vi "1g_v3.vi"() -> ()   [LabVIEW 2017]
uses:
  <vilib>/Instr/_visa.llb/VISA Configure Serial Port (Instr).vi
panel:
  in  "stop":bool
  out "return count 2":u32
  out "read buffer 2":string
  out "return count":u32
  out "read buffer":string
  in  "milliseconds":dbl=100.0 min=100.0
  out "XY Graph":cluster{dbl[], u16[]}(graph)
  out "VISA resource name out":refnum<visa-resource-name>
  in  "VISA resource name":refnum<visa-resource-name>="COM3" caption="Serial COM port"
  # "Partially working code"
  # "REAL TIME FIBER OPTIC TEMPERATURE MONITORING SYSTEM"
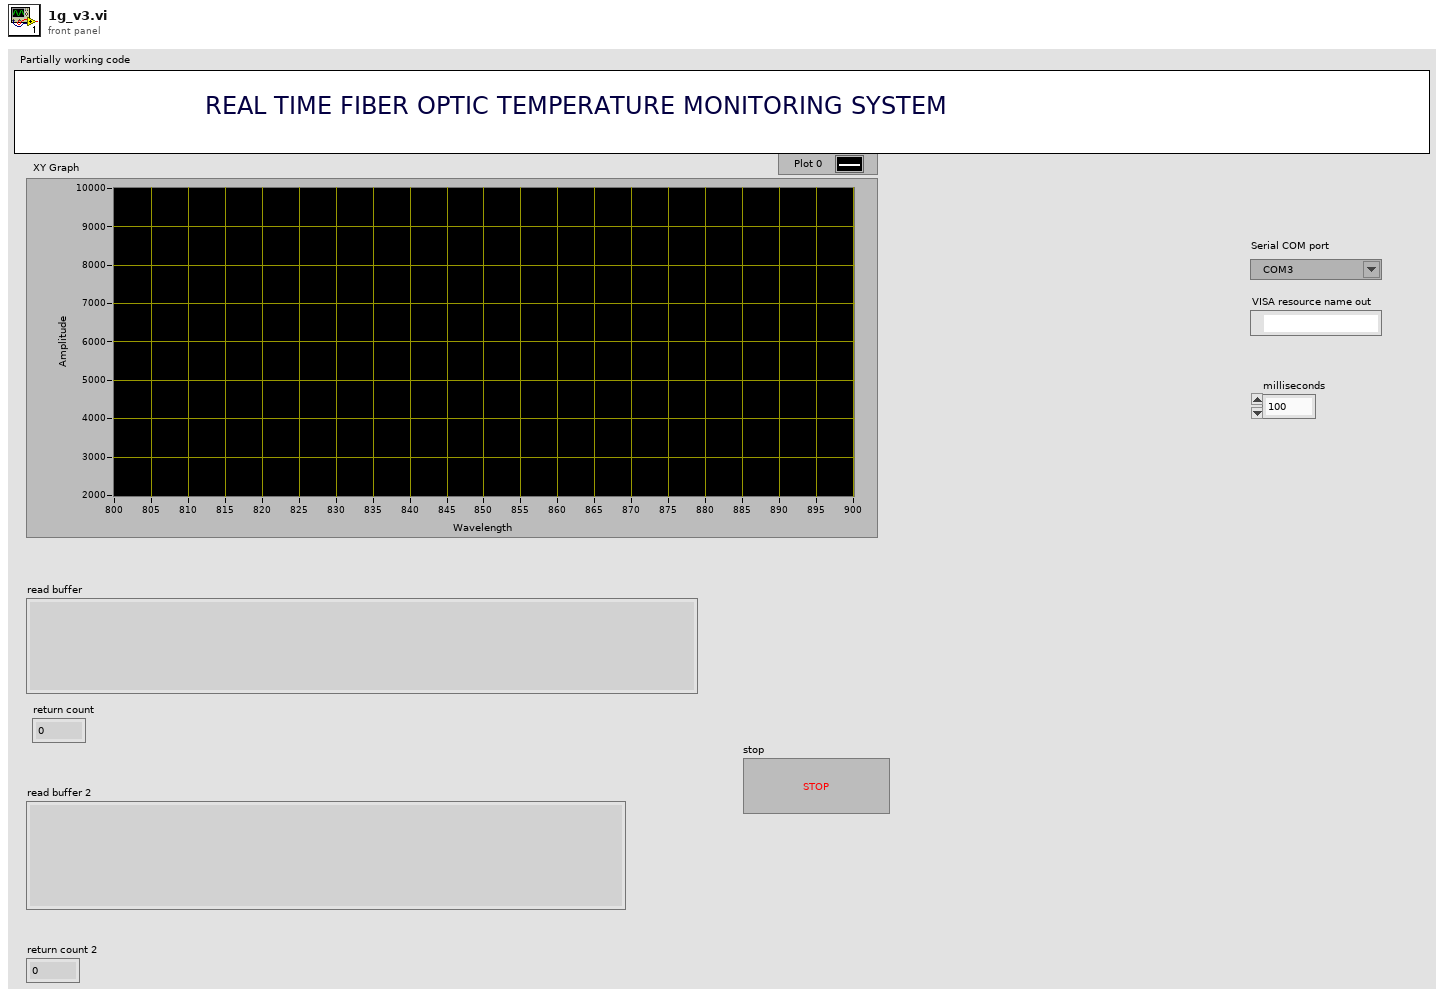
[diagram p1: front panel]
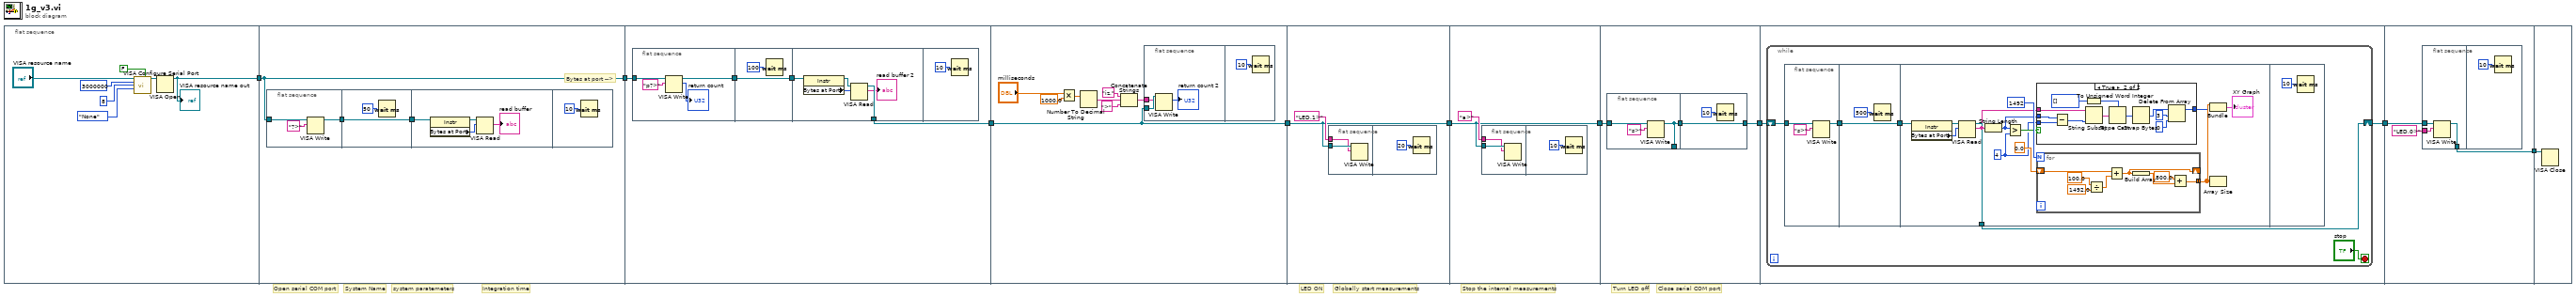
[diagram p0: block diagram]
diagram:
  # "Globally start measurements"
  # "LED ON"
  # "System Name"
  # "Integration time"
  # "system paratemeters"
  # "Close serial COM port"
  # "Turn LED off"
  # "Stop the internal measurements"
  # "Open serial COM port"
  n1 = flat-sequence {
    tunnel: [w10] -> w3
    tunnel: [w17] -> w9
    tunnel: w3 -> [w17]
    tunnel: w9 -> [w31]
    tunnel: [w30] -> w8
    tunnel: w8 -> [w49]
    tunnel: [w49] -> w7
    tunnel: w7 -> [w58]
    tunnel: [w58] -> w4
    tunnel: [w63] -> w2
    tunnel: w4 -> [w63]
    tunnel: w2 -> [w70]
    tunnel: [w68] -> w1
    tunnel: [w77] -> w6
    tunnel: w1 -> [w76]
    tunnel: w6 -> [w123]
    tunnel: [w122] -> w5
    tunnel: w5 -> [w129]
    frame #0 {
      n2 = call-poly "VISA Configure Serial Port"("VISA resource name"="VISA resource name", "Enable Termination\nChar (T)"=FALSE ("Enable Termination\nChar (T)"), "baud rate (9600)"=u32 3000000, "data bits (8)"=u16 8, "parity (0:none)"=enum16{"None", "Odd", "Even", "Mark", "Space"}."None") -> ("VISA resource name out"=w16:refnum<visa-resource-name>)  [unwired: 9 in, 1 out]
      n3 = VISA Open(VISA resource name=w16) -> (VISA resource name=w10:refnum<visa-resource-name>)  [unwired: 4 in, 1 out]
      "VISA resource name out" <- w10
    }
    frame #1 {
      # "Bytes at port -->"
      n4 = flat-sequence {
        tunnel: [w22] -> w19
        tunnel: w17 -> [w21]
        tunnel: [w23] -> w18
        tunnel: w19 -> [w23]
        tunnel: w18 -> [w28]
        frame #0 {
          n5 = VISA Write(VISA resource name=w21, write buffer="?>") -> (VISA resource name out=w22:refnum<visa-resource-name>)  [unwired: 1 in, 2 out]
        }
        frame #1 {
          n6 = Wait (ms)(milliseconds to wait=u32 50 ("Zu wartende ms")) -> ()  [unwired: 1 out]
        }
        frame #2 {
          n7 = property class="Instr"(reference=w28) -> (reference out=w27:refnum<visa-resource-name>, "Bytes at Port"=w26:u32)  [unwired: 1 in, 1 out]
          n8 = VISA Read(VISA resource name=w27, byte count=w26) -> (read buffer=→"read buffer":string)  [unwired: 1 in, 3 out]
        }
        frame #3 {
          n9 = Wait (ms)(milliseconds to wait=u32 10 ("Zu wartende ms")) -> ()  [unwired: 1 out]
        }
      }
    }
    frame #2 {
      n10 = flat-sequence {
        tunnel: [w37] -> w33
        tunnel: w31 -> [w35]
        tunnel: [w38] -> w32
        tunnel: w33 -> [w38]
        tunnel: w32 -> [w44]
        tunnel: [w41] -> w30
        frame #0 {
          n11 = VISA Write(VISA resource name=w35, write buffer="p?>") -> (VISA resource name out=w37:refnum<visa-resource-name>, return count=→"return count":u32)  [unwired: 1 in, 1 out]
        }
        frame #1 {
          n12 = Wait (ms)(milliseconds to wait=u32 100 ("Zu wartende ms")) -> ()  [unwired: 1 out]
        }
        frame #2 {
          n13 = property class="Instr"(reference=w44) -> (reference out=w43:refnum<visa-resource-name>, "Bytes at Port"=w42:u32)  [unwired: 1 in, 1 out]
          n14 = VISA Read(VISA resource name=w43, byte count=w42) -> (VISA resource name out=w41:refnum<visa-resource-name>, read buffer=→"read buffer 2":string)  [unwired: 1 in, 2 out]
        }
        frame #3 {
          n15 = Wait (ms)(milliseconds to wait=u32 10 ("Zu wartende ms")) -> ()  [unwired: 1 out]
        }
      }
    }
    frame #3 {
      n16 = Multiply(x="milliseconds", y=1000.0) -> (x*y=w46:dbl)
      n17 = Number To Decimal String(number=w46) -> (decimal integer string=w53:string)  [unwired: 1 in]
      n18 = Concatenate Strings("iz," ("String"), w53, ">" ("String")) -> (w50:string)
      n19 = flat-sequence {
        tunnel: w49 -> [w56]
        tunnel: w50 -> [w55]
        frame #0 {
          n20 = VISA Write(VISA resource name=w56, write buffer=w55) -> (return count=→"return count 2":u32)  [unwired: 1 in, 2 out]
        }
        frame #1 {
          n21 = Wait (ms)(milliseconds to wait=u32 10 ("Zu wartende ms")) -> ()  [unwired: 1 out]
        }
      }
    }
    frame #4 {
      n22 = flat-sequence {
        tunnel: w58 -> [w61]
        tunnel: "LED,1>" ("String") -> [w60]
        frame #0 {
          n23 = VISA Write(VISA resource name=w61, write buffer=w60) -> ()  [unwired: 1 in, 3 out]
        }
        frame #1 {
          n24 = Wait (ms)(milliseconds to wait=u32 20 ("Zu wartende ms")) -> ()  [unwired: 1 out]
        }
      }
    }
    frame #5 {
      n25 = flat-sequence {
        tunnel: w63 -> [w66]
        tunnel: "a>" ("String") -> [w65]
        frame #0 {
          n26 = VISA Write(VISA resource name=w66, write buffer=w65) -> ()  [unwired: 1 in, 3 out]
        }
        frame #1 {
          n27 = Wait (ms)(milliseconds to wait=u32 10 ("Zu wartende ms")) -> ()  [unwired: 1 out]
        }
      }
    }
    frame #6 {
      n28 = flat-sequence {
        tunnel: [w71] -> _
        tunnel: w70 -> [w72]
        tunnel: [w71] -> w69
        tunnel: [w75] -> w68
        tunnel: w69 -> [w75]
        frame #0 {
          n29 = VISA Write(VISA resource name=w72, write buffer="s>") -> (VISA resource name out=w71:refnum<visa-resource-name>)  [unwired: 1 in, 2 out]
        }
        frame #1 {
          n30 = Wait (ms)(milliseconds to wait=u32 10) -> ()  [unwired: 1 out]
        }
      }
    }
    frame #7 {
      n31 = while {
        shift-right: [w80] -> w77
        shift-left: w76 -> [w79]
        stop <- "stop" stop-if-true
        n32 = flat-sequence {
          tunnel: [w85] -> w82
          tunnel: w79 -> [w83]
          tunnel: [w86] -> w81
          tunnel: w82 -> [w86]
          tunnel: w81 -> [w95]
          tunnel: [w94] -> w80
          frame #0 {
            n33 = VISA Write(VISA resource name=w83, write buffer="s>") -> (VISA resource name out=w85:refnum<visa-resource-name>)  [unwired: 1 in, 2 out]
          }
          frame #1 {
            n34 = Wait (ms)(milliseconds to wait=u32 500 ("Zu wartende ms")) -> ()  [unwired: 1 out]
          }
          frame #2 {
            w88 = 4 ("y")
            n35 = property class="Instr"(reference=w95) -> (reference out=w93:refnum<visa-resource-name>, "Bytes at Port"=w92:u32)  [unwired: 1 in, 1 out]
            n36 = VISA Read(VISA resource name=w93, byte count=w92) -> (VISA resource name out=w94:refnum<visa-resource-name>, read buffer=w91:string)  [unwired: 1 in, 2 out]
            n37 = String Length(string=w91) -> (length=w90:i32)
            n38 = Greater?(x=w90, y=w88) -> (0:w89:bool)
            n39 = case shown="True" w89 {
              tunnel: w91 -> [_ w112]
              tunnel: w90 -> [_ w111]
              tunnel: w88 -> [_ w110]
              tunnel: [_ w101] -> w98
              frame False {
              }
              frame True {
                n40 = Subtract(x=w111, y=w110) -> (x-y=w109:i32)
                n41 = To Unsigned Word Integer(number=i32[] []) -> (unsigned 16bit integer=w108:u16[])
                n42 = String Subset(string=w112, length (rest)=w109) -> (substring=w107:string)  [unwired: 1 in]
                n43 = Type Cast(type=w108, x=w107) -> (*(type *) &x=w105:u16[])
                n44 = Swap Bytes(anything=w105) -> (byte swapped=w104:u16[])
                n45 = Delete From Array(array=w104, length=3, index=0) -> (array with subset deleted=w101:u16[])  [unwired: 1 out]
              }
            }
            n46 = for {
              N: 1492 -> [_]
              shift-right: [w119] -> _
              shift-left: 0.0 -> [w120]
              tunnel: [w116] -> w100 mode=concatenating
              n47 = Divide(x=100.0 ("x/y"), y=1492.0) -> (x/y=w113:dbl)
              n48 = Add(x=w120, y=w113) -> (x+y=w119:dbl)
              n49 = Build Array(w119) -> (w117:dbl[])
              n50 = Add(x=800.0 ("x+y"), y=w117) -> (x+y=w116:dbl[])
            }
            n51 = Bundle(w100, w98) -> (→"XY Graph":cluster{dbl[], u16[]})  [unwired: 1 in]
            n52 = Array Size(array=w100) -> ()  [unwired: 1 out]
          }
          frame #3 {
            n53 = Wait (ms)(milliseconds to wait=u32 10 ("Zu wartende ms")) -> ()  [unwired: 1 out]
          }
        }
      }
    }
    frame #8 {
      n54 = flat-sequence {
        tunnel: w123 -> [w127]
        tunnel: "LED,0>" ("String") -> [w126]
        tunnel: [w125] -> w122
        frame #0 {
          n55 = VISA Write(VISA resource name=w127, write buffer=w126) -> (VISA resource name out=w125:refnum<visa-resource-name>)  [unwired: 1 in, 2 out]
        }
        frame #1 {
          n56 = Wait (ms)(milliseconds to wait=u32 10 ("Zu wartende ms")) -> ()  [unwired: 1 out]
        }
      }
    }
    frame #9 {
      n57 = VISA Close(VISA resource name=w129) -> ()  [unwired: 1 in, 1 out]
    }
  }
